vi "VIH HelpGen - Build - Externals.vi"(8 "error in":errorcluster, 9 "File paths":path[](array[path]), 10 "Items":T2, 11 "Project Tree":T1) -> (0 "error out":errorcluster, 2 "Items out":T2, 3 "dup Project Tree":T1)   [LabVIEW 2014]
doc: "::: VI Helpeks :::\nCopyright (c) 2000-2026 Konstantin Shifershteyn. All rights reserved."
uses:
  _VIH Project Manager.llb/VIH Project Tree Typedef - Tree Refnum.ctl
panel:
  # "VI Helpeks\nCopyright (c) 2012-2026 Konstantin Shifershteyn"
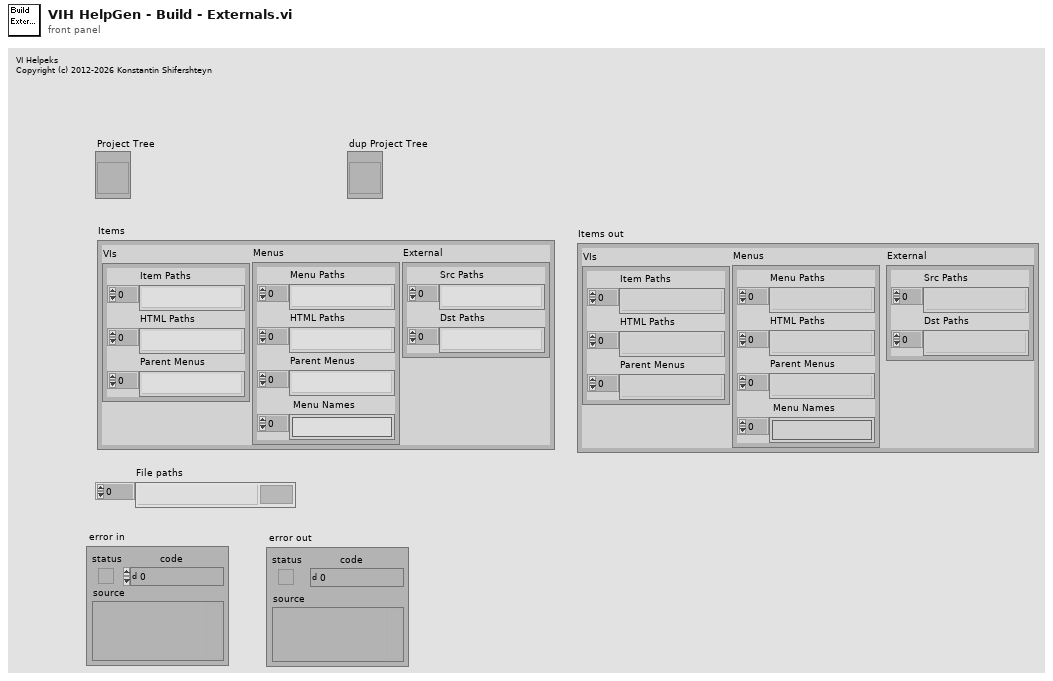
[diagram p1: front panel]
types:
  T1 = typedef "VIH Project Tree Typedef - Tree Refnum.ctl" = refnum<vi>
  T2 = cluster{"VIs":cluster{"Item Paths":path[], "HTML Paths":path[], "Parent Menus":path[]}, "Menus":cluster{"Menu Paths":path[], "HTML Paths":path[], "Parent Menus":path[], " Menu Names":string[]}, "External":cluster{"Src Paths":path[], "Dst Paths":path[]}}
  T3 = enum16{"nop", "Start", "Stop", "Run-prep", "Run-VI", "Run-Menu"}
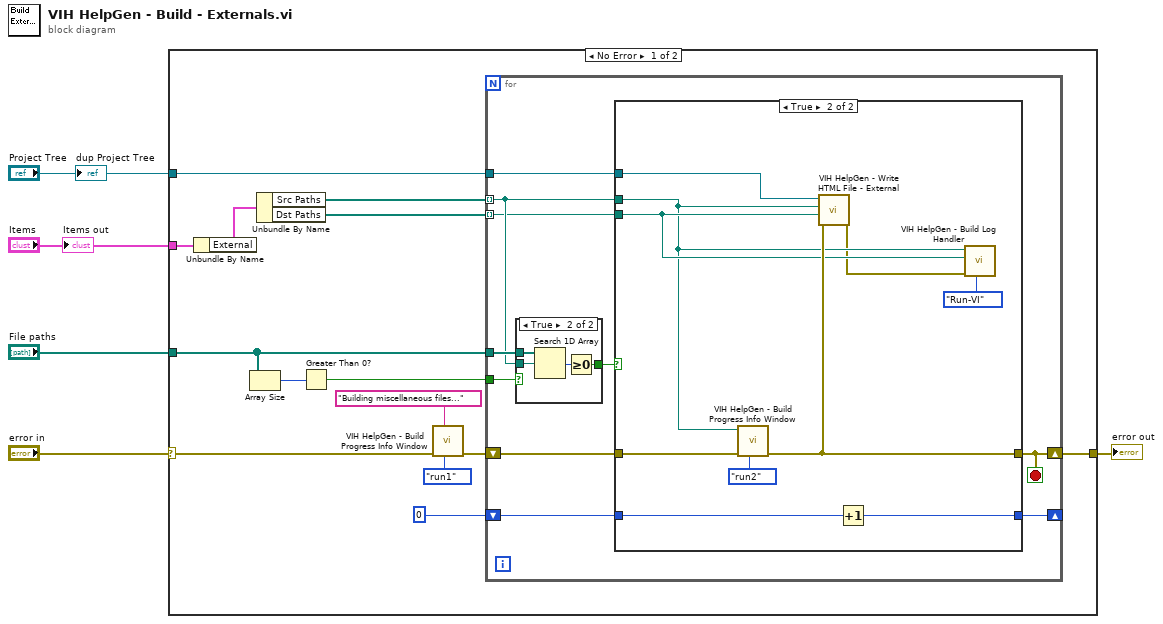
[diagram p0: block diagram]
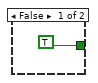
[diagram p3: hidden frame]
diagram:
  n1 = case shown="No Error" "error in" {
    selector: "error in" -> [w6 w47]
    tunnel: "File paths" -> [w19 _]
    tunnel: [w17 w47] -> w4
    tunnel: "Items" -> [w15 _]
    tunnel: "Project Tree" -> [w7 _]
    frame No Error {
      n2 = Unbundle By Name(w15) -> ("External"=w16:cluster{"Src Paths":path[], "Dst Paths":path[]})
      n3 = Array Size(array=w19) -> (size(s)=w9:i32)
      n4 = Unbundle By Name(w16) -> ("Src Paths"=w8:path[], "Dst Paths"=w18:path[])
      n5 = Greater Than 0?(x=w9) -> (x > 0?=w10:bool)
      n6 = call "VIH HelpGen - Build Progress Info Window.vi"("Mode (run1)"=enum16{"start", "stop", "run1", "run2"}."run1" ("Mode (run)"), "Message"="Building miscellaneous files...", "error in"=w6) -> ("error out"=w14:errorcluster)  [unwired: 8 in]
      n7 = for {
        tunnel: w10 -> [w29]
        tunnel: w19 -> [w28]
        tunnel: w8 -> [w26] mode=indexing
        tunnel: w18 -> [w25] mode=indexing
        shift-right: [w20] -> w17
        shift-left: w14 -> [w24]
        shift-right: [w22] -> _
        shift-left: 0 -> [w23]
        tunnel: w7 -> [w21]
        stop <- w20 stop-if-true
        n8 = case shown="True" w29 {
          tunnel: w28 -> [_ w46]
          tunnel: w26 -> [_ w45]
          tunnel: [TRUE w43] -> w27
          frame False {
          }
          frame True {
            n9 = Search 1D Array(1D array=w46, element=w45) -> (index of element=w44:i32)  [unwired: 1 in]
            n10 = Greater Or Equal To 0?(x=w44) -> (x >= 0?=w43:bool)
          }
        }
        n11 = case shown="True" w27 {
          tunnel: w26 -> [_ w33]
          tunnel: w25 -> [_ w34]
          tunnel: w24 -> [w31 w40]
          tunnel: [w31 w35] -> w20
          tunnel: w23 -> [w30 w39]
          tunnel: [w30 w38] -> w22
          tunnel: w21 -> [_ w37]
          frame False {
          }
          frame True {
            n12 = call "VIH HelpGen - Build Progress Info Window.vi"("Mode (run1)"=enum16{"start", "stop", "run1", "run2"}."run2" ("Mode (run)"), "error in"=w40, "Cur path"=w33) -> ("error out"=w35:errorcluster)  [unwired: 8 in]
            n13 = call "VIH HelpGen - Write HTML File - External.vi"("error in"=w35, "Destination Path"=w34, "Source Path"=w33, "Project Tree"=w37) -> ("error out"=w32:errorcluster)  [unwired: 6 in, 1 out]
            n14 = Increment(x=w39) -> (x+1=w38:i32)
            n15 = call "VIH HelpGen - Build Log Handler.vi"("cmd (nop)"=T3."Run-VI" ("cmd"), "error in"=w32, "Out File Path"=w34, "Src File Path"=w33) -> ()  [unwired: 3 in, 5 out]
          }
        }
      }
    }
    frame Error {
    }
  }
  "error out" <- w4
  "Items out" <- "Items"
  "dup Project Tree" <- "Project Tree"
